vi "Digital_Read_Ex.vi"() -> ()   [LabVIEW 2026]
panel:
  in  "VISA resource name":refnum<visa-resource-name>
  in  "Stop Button":bool
  out "Out":bool
  in  "Canal Read":u8
  out "error out":errorcluster
  # "Ejemplo: Digital Read"
  # "Descripción: Lee el estado de un pin digital del microcontrolador y lo muestra en un indicador."
  # "Configuracion"
  # "Indicadores"
  # "Control"
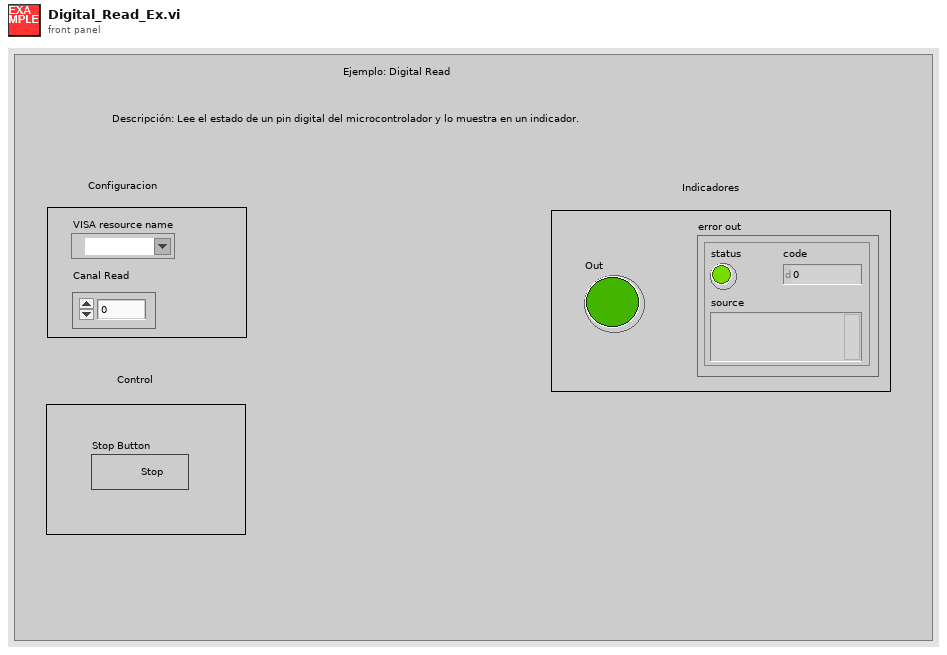
[diagram p1: front panel]
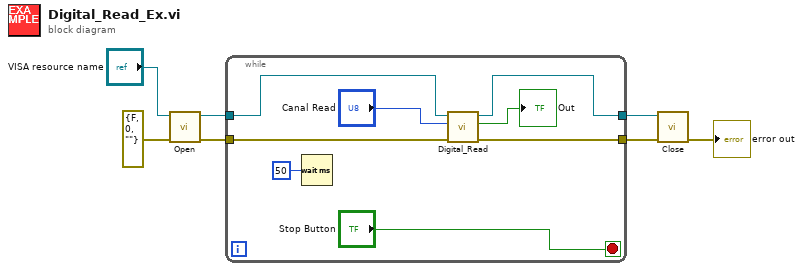
[diagram p0: block diagram]
diagram:
  n1 = call "Open.vi"("error in (no error)"=errorcluster {"status"=FALSE, "code"=0, "source"=""}, "VISA resource name"="VISA resource name") -> ("error out"=w7:errorcluster, "VISA resource name out"=w3:refnum<visa-resource-name>)  [unwired: 8 in]
  n2 = while {
    tunnel: w7 -> [w13]
    tunnel: w3 -> [w14]
    tunnel: [w9] -> w2
    tunnel: [w8] -> w1
    stop <- "Stop Button" stop-if-true
    n3 = Wait (ms)(milliseconds to wait=u32 50) -> ()  [unwired: 1 out]
    n4 = call "Digital_Read.vi"("error in (no error)"=w13, "Canal"="Canal Read", "VISA resource name"=w14) -> ("error out"=w8:errorcluster, "Out"=→"Out":bool, "VISA resource name out"=w9:refnum<visa-resource-name>)  [unwired: 6 in]
  }
  n5 = call "Close.vi"("error in (no error)"=w1, "VISA resource name"=w2) -> ("error out"=→"error out":errorcluster)  [unwired: 9 in]
